vi "NR Call Check.vi"(8 "error in (no error)":errorcluster caption="에러 입력(에러 없음)", 11 "Instrument Manager 입력":refnum<class "Instrument Manager.lvclass">) -> (0 "error out":errorcluster caption="에러 출력", 2 "Connected?":bool, 3 "Instrument Manager 출력":refnum<class "Instrument Manager.lvclass">)   [LabVIEW 2023, in "Instrument Manager.lvclass"]
uses:
  Instrument Manager.lvclass
  Module/ANRITSU Call Box/Type Definition/Call Processing Status Enum.ctl
  Instrument Manager.lvclass/Instrument Manager.ctl
  Module/ANRITSU Call Box/Interface Class/Anritsu Call Box.lvclass
  Module/ANRITSU Call Box/ANRITSU Call Box.lvlib
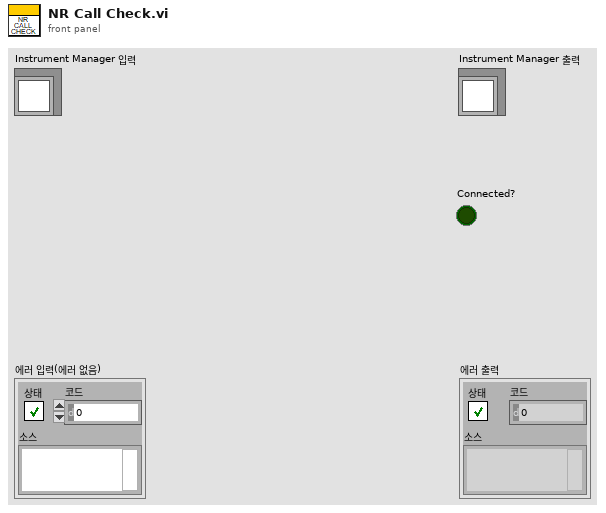
[diagram p1: front panel]
types:
  T1 = typedef "ANRITSU Call Box.lvlib/Call Processing Status Enum.ctl" = enum16{"Off", "Idle", "Idle (Regist)", "Registration", "UE Origination", "NW Origination", "Connected", "SCG Adding", "Connected (NSA)", "SCG Release", "Undefined1", "Undefined2", "Undefined3", "Handover", "NW Release", "UE Release", "Detach", "Setup", "Redirection"}
  T2 = cluster{"Anritsu Call Box":refnum<class "Anritsu Call Box.lvclass">, "Spectrum Analyzer":refnum<class "Interface_Spectrum.lvclass">, "RF Switch Box":refnum<class "RF Filter Box.lvclass">, "Turn Table":refnum<class "Interface - Turn Table.lvclass">, "Mast":refnum<class "Interface - Mast.lvclass">, "3D Controller":refnum<class "Interface_3D Controller.lvclass">}
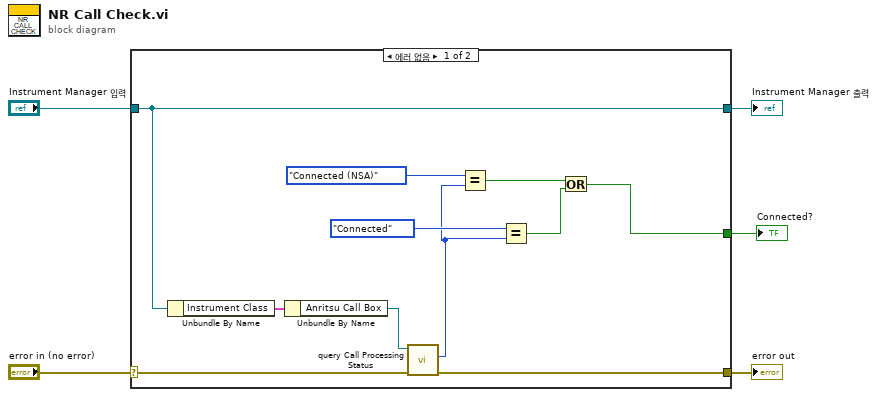
[diagram p0: block diagram]
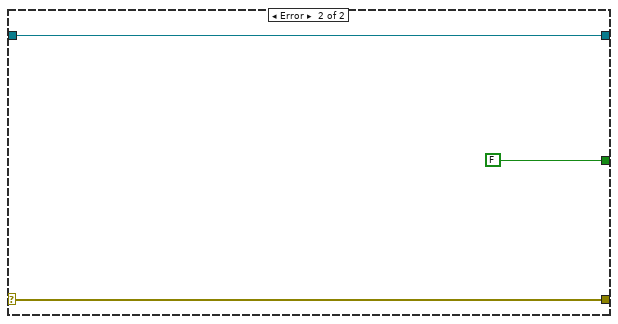
[diagram p2: hidden frame]
diagram:
  n1 = case shown="에러 없음" "error in (no error)" {
    selector: "error in (no error)" -> [w13 w19]
    tunnel: [w11 w19] -> w4
    tunnel: [w16 w18] -> w2
    tunnel: "Instrument Manager 입력" -> [w16 w18]
    tunnel: [w6 FALSE] -> w1
    frame No Error {
      n2 = Unbundle By Name(w16) -> ("Instrument Class"=w15:T2)
      n3 = Unbundle By Name(w15) -> ("Anritsu Call Box"=w14:refnum<class "Anritsu Call Box.lvclass">)
      n4 = call-dynamic "query Call Processing Status.vi"("error in (no error)"=w13, "Anritsu Call Box in"=w14) -> ("error out"=w11:errorcluster, "Call Processing Status"=w8:T1)  [unwired: 7 in, 1 out]
      n5 = Equal?(x=Call_Processing_Status_Enum."Connected (NSA)" ("Call Processing Status"), y=w8) -> (x = y?=w9:bool)
      n6 = Equal?(x=Call_Processing_Status_Enum."Connected" ("Call Processing Status"), y=w8) -> (x = y?=w7:bool)
      n7 = Or(x=w9, y=w7) -> (x .or. y?=w6:bool)
    }
    frame Error {
    }
  }
  "error out" <- w4
  "Instrument Manager 출력" <- w2
  "Connected?" <- w1
